vi "Test Deserialize Variants.vi"(8 "error in (no error)":errorcluster) -> (0 "error out":errorcluster)   [LabVIEW 2013]
uses:
  src/Deserializer/JSON Deserializer/JSON Deserializer.lvclass
  <userlib>/_OpenG.lib/lvdata/lvdata.llb/Array of VData to VCluster__ogtk.vi
  <vilib>/addons/_JKI Toolkits/Caraya/classes/Test/Test.lvclass
  <vilib>/addons/_JKI Toolkits/Caraya/classes/Assert/Assert.lvclass
  src/JKI JSON Serialization.lvlib
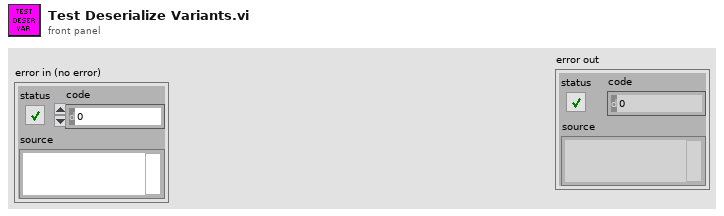
[diagram p1: front panel]
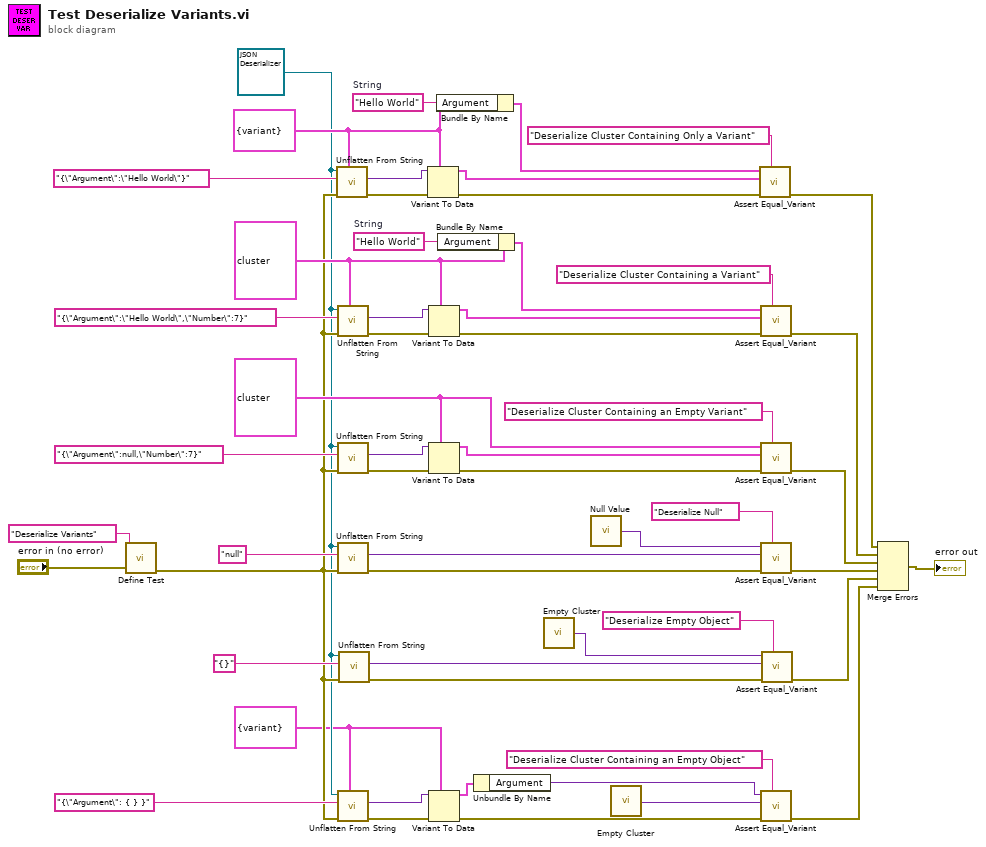
[diagram p0: block diagram]
diagram:
  w1 = cluster{"Argument":variant} {"Argument"=variant}
  w20 = cluster{"Argument":variant, "Number":i32} {"Argument"=variant, "Number"=7}
  w31 = "Hello World"  # String
  w34 = cluster{"Argument":variant} {"Argument"=variant}
  w44 = "Hello World"  # String
  w41 = cluster{"Argument":variant, "Number":i32} {"Argument"=variant, "Number"=7}
  w8 = refnum<class "JSON Deserializer.lvclass"> refnum ("Deserializer out")
  n1 = call <vilib>:"Define Test.vi"("error in (no error)"="error in (no error)", "Label (VI Title)"="Deserialize Variants") -> ("error out"=w9:errorcluster)  [unwired: 9 in]
  n2 = call-dynamic "Unflatten From String.vi"("Type and Defaults"=w34, "error in (no error)"=w9, "String"="{\"Argument\":\"Hello World\"}", "Deserializer in"=w8) -> ("error out"=w33:errorcluster, "Variant"=w32:variant)  [unwired: 5 in, 1 out]
  n3 = call-dynamic "Unflatten From String.vi"("Type and Defaults"=w41, "error in (no error)"=w9, "String"="{\"Argument\":\"Hello World\",\"Number\":7}", "Deserializer in"=w8) -> ("error out"=w42:errorcluster, "Variant"=w43:variant)  [unwired: 5 in, 1 out]
  n4 = call-dynamic "Unflatten From String.vi"("error in (no error)"=w9, "String"="{\"Argument\":null,\"Number\":7}", "Deserializer in"=w8) -> ("error out"=w25:errorcluster, "Variant"=w24:variant)  [unwired: 6 in, 1 out]
  n5 = call-dynamic "Unflatten From String.vi"("error in (no error)"=w9, "String"="null", "Deserializer in"=w8) -> ("error out"=w49:errorcluster, "Variant"=w48:variant)  [unwired: 6 in, 1 out]
  n6 = call-dynamic "Unflatten From String.vi"("Type and Defaults"=w1, "error in (no error)"=w9, "String"="{\"Argument\": { } }", "Deserializer in"=w8) -> ("error out"=w13:errorcluster, "Variant"=w12:variant)  [unwired: 5 in, 1 out]
  n7 = call-dynamic "Unflatten From String.vi"("error in (no error)"=w9, "String"="{}", "Deserializer in"=w8) -> ("error out"=w17:errorcluster, "Variant"=w16:variant)  [unwired: 6 in, 1 out]
  n8 = Variant To Data(error in=w33, type=w34, Variant=w32) -> (data=w35:cluster{"Argument":variant}, error out=w37:errorcluster)
  n9 = Variant To Data(error in=w42, type=w41, Variant=w43) -> (data=w40:cluster{"Argument":variant, "Number":i32}, error out=w38:errorcluster)
  n10 = Variant To Data(error in=w25, type=w20, Variant=w24) -> (data=w26:cluster{"Argument":variant, "Number":i32}, error out=w27:errorcluster)
  n11 = Variant To Data(error in=w13, type=w1, Variant=w12) -> (data=w5:cluster{"Argument":variant}, error out=w14:errorcluster)
  n12 = Bundle By Name(cluster=w34, "Argument"=w31) -> (w36:cluster{"Argument":variant})
  n13 = Bundle By Name(cluster=w41, "Argument"=w44) -> (w39:cluster{"Argument":variant, "Number":i32})
  n14 = Unbundle By Name(w5) -> ("Argument"=w4:variant)
  n15 = call "Empty Cluster.vi"() -> ("Empty Cluster"=w2:variant)
  n16 = call "Null Value.vi"() -> ("Null"=w6:variant)
  n17 = call "Empty Cluster.vi"() -> ("Empty Cluster"=w3:variant)
  n18 = call <vilib>:"Assert Equal_Variant.vi"("Label"="Deserialize Cluster Containing Only a Variant", "error in (no error)"=w37, "Y"=w35, "X"=w36) -> ("error out"=w28:errorcluster)  [unwired: 7 in]
  n19 = call <vilib>:"Assert Equal_Variant.vi"("Label"="Deserialize Cluster Containing a Variant", "error in (no error)"=w38, "Y"=w40, "X"=w39) -> ("error out"=w46:errorcluster)  [unwired: 7 in]
  n20 = call <vilib>:"Assert Equal_Variant.vi"("Label"="Deserialize Cluster Containing an Empty Variant", "error in (no error)"=w27, "Y"=w26, "X"=w20) -> ("error out"=w21:errorcluster)  [unwired: 7 in]
  n21 = call <vilib>:"Assert Equal_Variant.vi"("Label"="Deserialize Null", "error in (no error)"=w49, "Y"=w48, "X"=w6) -> ("error out"=w52:errorcluster)  [unwired: 7 in]
  n22 = call <vilib>:"Assert Equal_Variant.vi"("Label"="Deserialize Cluster Containing an Empty Object", "error in (no error)"=w14, "Y"=w3, "X"=w4) -> ("error out"=w7:errorcluster)  [unwired: 7 in]
  n23 = call <vilib>:"Assert Equal_Variant.vi"("Label"="Deserialize Empty Object", "error in (no error)"=w17, "Y"=w16, "X"=w2) -> ("error out"=w15:errorcluster)  [unwired: 7 in]
  n24 = Merge Errors(w28, w46, w21, w52, w15, w7) -> (→"error out":errorcluster)
